vi "Grab Image.vi"(8 "error in (no error)":errorcluster, 11 "Refnum in":T1) -> (0 "error out":errorcluster, 2 "displayTime":u32, 3 "Refnum out":T1)   [LabVIEW 2025, in "VarexWrapper.lvlib"]
uses:
  VarexWrapper.lvlib
  <vilib>/vision/Image Controls.llb/IMAQ Image.ctl
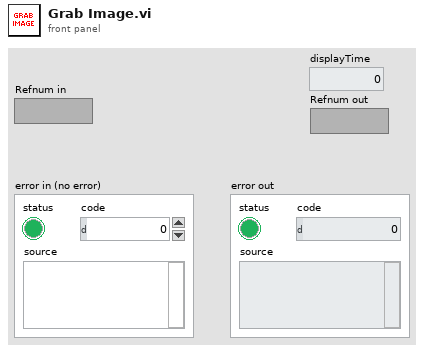
[diagram p1: front panel]
types:
  T1 = typedef "IMAQ Image.ctl" = refnum<image>
  T2 = enum32{"Map Pixel Pointer", "Unmap Pixel Pointer", "Get Pixels Infos"}
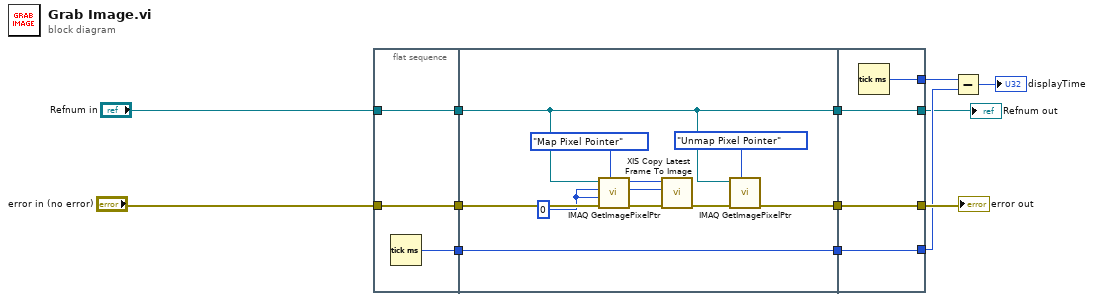
[diagram p0: block diagram]
diagram:
  n1 = flat-sequence {
    tunnel: "error in (no error)" -> [w15]
    tunnel: "Refnum in" -> [w16]
    tunnel: [w16] -> w10
    tunnel: [w15] -> w9
    tunnel: [w14] -> w6
    tunnel: w10 -> [w17]
    tunnel: w9 -> [w26]
    tunnel: [w27] -> w8
    tunnel: [w18] -> w7
    tunnel: w6 -> [w18]
    tunnel: [w17] -> w2
    tunnel: [w31] -> w13
    tunnel: w8 -> [w31]
    tunnel: w7 -> [w29]
    tunnel: [w30] -> w5
    tunnel: [w29] -> w4
    tunnel: [w28] -> w1
    tunnel: w2 -> [w28]
    frame #0 {
      n2 = Tick Count (ms)() -> (millisecond timer value=w14:u32)
    }
    frame #1 {
      w25 = 0 ("X Coordinate")
      n3 = call "IMAQ GetImagePixelPtr"("Function"=T2."Map Pixel Pointer", "error in (no error)"=w26, "Y Coordinate"=w25, "X Coordinate"=w25, "Image"=w17) -> ("error out"=w19:errorcluster, "LineWidth(Pixels)"=w21:i32, "Pixel Pointer out"=w22:u64)  [unwired: 1 in, 3 out]
      n4 = call "XIS Copy Latest Frame To Image.vi"("error in (no error)"=w19, "LVLineWidthPixels"=w21, "LVImagePtr"=w22) -> ("error out"=w20:errorcluster)  [unwired: 7 in, 1 out]
      n5 = call "IMAQ GetImagePixelPtr"("Function"=T2."Unmap Pixel Pointer", "error in (no error)"=w20, "Image"=w17) -> ("error out"=w27:errorcluster)  [unwired: 3 in, 5 out]
    }
    frame #2 {
      n6 = Tick Count (ms)() -> (millisecond timer value=w30:u32)
    }
  }
  n7 = Subtract(x=w5, y=w4) -> (x-y=→"displayTime":u32)
  "error out" <- w13
  "Refnum out" <- w1
